vi "CE Client - Var Bridge.vi"(7 "local VC Handle":T1=-1, 8 "error in":errorcluster, 9 "direction":enum16{"client to srv", "srv to client"}(ring), 10 "var name":string, 11 "CE session":T4={"VI refnum"=refnum, "VC Handle"=-1}) -> (0 "error out":errorcluster, 2 "values out":T3={"type"=enum."DBL Number", "dbl"=0.0, "cdb"=0.0+0.0i, "str"="", "1d dbl"=[], "1d cdb"=[], "1d str"=[], "2d dbl"=[], "2d cdb"=[], "2d str"=[]} {"2d cdb" format="%.2f"; "2d dbl" format="%.2f"; "1d cdb" format="%.2f"; "1d dbl" format="%.2f"; "cdb" format="%.2f"; "dbl" format="%.2f"}, 3 "dup CE session":T4={"VI refnum"=refnum, "VC Handle"=-1}, 5 "dup local VC Handle":T1=-1)   [LabVIEW 2021]
doc: "::: CalcExpress Toolkit :::\nCopyright (c) 2000-2026 Konstantin Shifershteyn. All rights reserved."
uses:
  CE Session.ctl
  vi.lib/addons/CalcExpress/cetypes.llb/VarMan Variable Context Handle.ctl
  vi.lib/addons/CalcExpress/cetypes.llb/CalcExpress Data Type.ctl
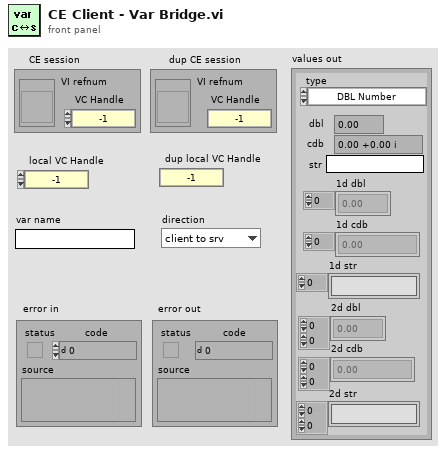
[diagram p1: front panel]
types:
  T1 = typedef "VarMan Variable Context Handle.ctl" = i32
  T2 = typedef "CalcExpress Data Type.ctl" = enum32{"String", "DBL Number", "identifier", "1D Array of DBL", "2D Array of DBL", "CDB Number", "1D Array of CDB", "2D Array of CDB", "1D Array of String", "2D Array of String", "Unknown data type"}
  T3 = cluster{"type":T2, "dbl":dbl, "cdb":cdb, "str":string, "1d dbl":dbl[], "1d cdb":cdb[], "1d str":string[], "2d dbl":dbl[][], "2d cdb":cdb[][], "2d str":string[][]}
  T4 = typedef "CE Session.ctl" = cluster{"VI refnum":refnum<vi>, "VC Handle":T1}
  T5 = cluster{"type":enum32{"String", "DBL Number", "identifier", "1D Array of DBL", "2D Array of DBL", "CDB Number", "1D Array of CDB", "2D Array of CDB", "1D Array of String", "2D Array of String", "Unknown data type"}, "dbl":dbl, "cdb":cdb, "str":string, "1d dbl":dbl[], "1d cdb":cdb[], "1d str":string[], "2d dbl":dbl[][], "2d cdb":cdb[][], "2d str":string[][]}
  T6 = enum16{"create", "destroy", "set value", "get value"}
  T7 = enum16{"open session", "close session", "CalcExpress", "VarMan", "VarMan (low level)"}
  T8 = enum32{"String", "DBL Number", "identifier", "1D Array of DBL", "2D Array of DBL", "CDB Number", "1D Array of CDB", "2D Array of CDB", "1D Array of String", "2D Array of String", "Unknown data type"}
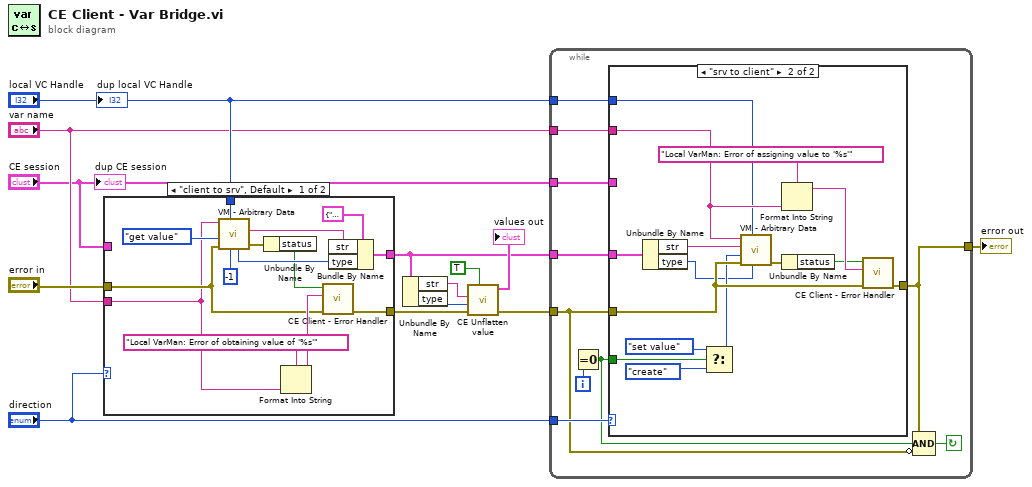
[diagram p0: block diagram]
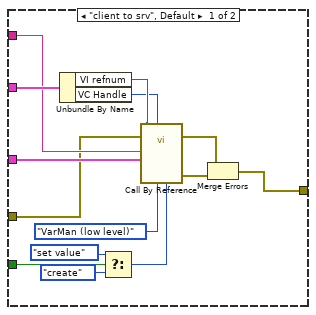
[diagram p2: hidden frame]
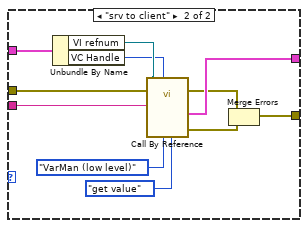
[diagram p3: hidden frame]
diagram:
  n1 = case shown="\"client to srv\", Default" "direction" {
    tunnel: "error in" -> [w17 w33]
    tunnel: "local VC Handle" -> [w19 _]
    tunnel: [w25 w30] -> w5
    tunnel: [w27 w38] -> w6
    tunnel: "var name" -> [w14 w29]
    tunnel: "CE session" -> [_ w28]
    frame "client to srv", Default {
      n2 = call "VM - Arbitrary Data.vi"("var type"=-1, "VC Handle"=w19, "error in"=w17, "cmd"=T6."get value", "name_spec"=w14) -> ("error out"=w23:errorcluster, "flattened value out"=w21:string, "var type out"=w22:u32)  [unwired: 1 in, 3 out]
      n3 = Unbundle By Name(w23) -> ("status"=w20:bool)
      n4 = Format Into String(format string="Local VarMan: Error of obtaining value of '%s'" ("CE error message"), w14) -> (resulting string=w24:string)  [unwired: 2 in, 1 out]
      n5 = call "CE Client - Error Handler.vi"("error before"=w17, "error message"=w24, "CE error status"=w20) -> ("error out"=w25:errorcluster)  [unwired: 6 in]
      n6 = Bundle By Name(cluster=T5 {"type"=enum."DBL Number", "dbl"=0.0, "cdb"=0.0+0.0i, "str"="", "1d dbl"=[], "1d cdb"=[], "1d str"=[], "2d dbl"=[], "2d cdb"=[], "2d str"=[]} ("values out"), "str"=w21, "type"=w22) -> (w27:T5)
    }
    frame "srv to client" {
      n7 = Unbundle By Name(w28) -> ("VI refnum"=w35:refnum<vi>, "VC Handle"=w34:T1)
      n8 = call-by-ref "?"(reference=w35, error in=w33, "var cmd"=T6."get value", "exec"=T7."VarMan (low level)", "VC Handle"=w34, "expression/name"=w29) -> (error out=w32:errorcluster, "error out"=w31:errorcluster, "values out"=w38:T5)  [unwired: 5 in, 2 out]
      n9 = Merge Errors(w32, w31) -> (w30:errorcluster)
    }
  }
  n10 = Unbundle By Name(w6) -> ("str"=w7:string, "type"=w8:T8)
  n11 = call "CE Unflatten value.vi"("Flattened DBL?"=TRUE, "error in"=w5, "type"=w8, "flattened data"=w7) -> ("error out"=w4:errorcluster, "values out"=→"values out":T3)  [unwired: 4 in]
  n12 = while {
    tunnel: "local VC Handle" -> [w43]
    tunnel: [w39] -> w10
    tunnel: "var name" -> [w44]
    tunnel: "CE session" -> [w45]
    tunnel: w6 -> [w46]
    tunnel: w4 -> [w40]
    tunnel: "direction" -> [w48]
    i -> [w47]
    stop <- w42 continue-if-true
    n13 = Equal To 0?(x=w47) -> (x = 0?=w41:bool)
    n14 = case shown="\"srv to client\"" w48 {
      tunnel: w40 -> [w52 w67]
      tunnel: w46 -> [w60 w75]
      tunnel: w45 -> [w59 _]
      tunnel: w44 -> [w58 w72]
      tunnel: w41 -> [w56 w76]
      tunnel: [w49 w74] -> w39
      tunnel: w43 -> [_ w71]
      frame "client to srv", Default {
        n15 = Unbundle By Name(w59) -> ("VI refnum"=w62:refnum<vi>, "VC Handle"=w61:T1)
        n16 = Select(t=T6."set value", s=w56, f=T6."create" ("var cmd")) -> (s? t:f=w53:T6)
        n17 = call-by-ref "?"(reference=w62, error in=w52, "var cmd"=w53, "exec"=T7."VarMan (low level)", "VC Handle"=w61, "values in"=w60, "expression/name"=w58) -> (error out=w50:errorcluster, "error out"=w51:errorcluster)  [unwired: 4 in, 3 out]
        n18 = Merge Errors(w50, w51) -> (w49:errorcluster)
      }
      frame "srv to client" {
        n19 = Unbundle By Name(w75) -> ("str"=w70:string, "type"=w63:T8)
        n20 = Select(t=T6."set value" ("cmd"), s=w76, f=T6."create" ("cmd")) -> (s? t:f=w66:T6)
        n21 = call "VM - Arbitrary Data.vi"("var type"=w63, "VC Handle"=w71, "error in"=w67, "cmd"=w66, "flattened value"=w70, "name_spec"=w72) -> ("error out"=w64:errorcluster)  [unwired: 5 out]
        n22 = Format Into String(format string="Local VarMan: Error of assigning value to '%s'", w72) -> (resulting string=w73:string)  [unwired: 2 in, 1 out]
        n23 = Unbundle By Name(w64) -> ("status"=w65:bool)
        n24 = call "CE Client - Error Handler.vi"("error before"=w67, "error message"=w73, "CE error status"=w65) -> ("error out"=w74:errorcluster)  [unwired: 6 in]
      }
    }
    n25 = Compound Arithmetic op=AND(w39, w41, invert w40) -> (w42:bool)
  }
  "error out" <- w10
  "dup CE session" <- "CE session"
  "dup local VC Handle" <- "local VC Handle"
